vi "CalcExpress.vi"(5 "directives":T1={"enaNamedConst"=TRUE}, 7 "VC Handle":T5=-1, 8 "error in":bool, 9 "params":T3={"autoVar"=TRUE, "enCpx"=TRUE}, 10 "repeat (1)":i32=1, 11 "expression":string) -> (0 "error out":bool, 1 "value type":T4=enum."DBL Number", 2 "string value":string, 3 "numeric value":dbl, 4 "error description":string)   [LabVIEW 2021]
doc: "The VI evaluates CalcExpress expressions and sequential scripts. To process non-sequential scripts involving loops and branches, use CSE VIs.\n\n<B>VC Handle</B> should contain handle of variable context. Variables of the corresponding context can be used in an expression.\n\n<B>repeat</B> control determines number of times an expression needs to be evaluated. By default, it is equal to one (1).\n\n<B>params</B> cluster specifies optional parameters influencing on evaluation.\n params.autoVar - If it's TRUE (by default) and there is a reference to unexistent variable on the left side of an assignment operator, CalcExpress implicitly creates the variable. If it's FALSE, all variables referenced in a script must be explicitly created either before or during evaluation.\n params.enCpx parameter enables or disables performing operators on operands of non-Numeric types (TRUE by default).\n\nFor more information, see help for this VI.\n\n::: CalcExpress Toolkit :::\nCopyright (c) 2000-2026 Konstantin Shifershteyn. All rights reserved."
uses:
  cetypes.llb/VarMan Variable Context Handle.ctl
  cetypes.llb/CalcExpress Data Type.ctl
  cetypes.llb/CalcExpress Execution Options.ctl
  cetypes.llb/CalcExpress Instance RefNum.ctl
  cetypes.llb/CalcExpress Parsing Directives.ctl
  cersrc/celveng32.dll
panel:
  in  "CE InstanceRef":T2
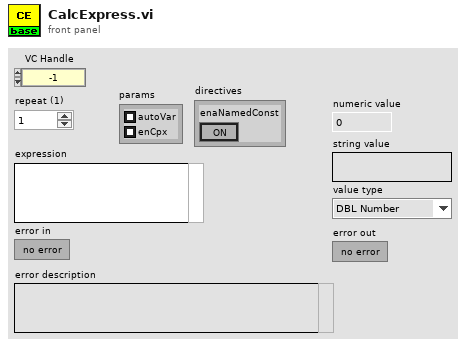
[diagram p1: front panel]
types:
  T1 = typedef "CalcExpress Parsing Directives.ctl" = cluster{"enaNamedConst":bool}
  T2 = typedef "CalcExpress Instance RefNum.ctl" = refnum<k1>
  T3 = typedef "CalcExpress Execution Options.ctl" = cluster{"autoVar":bool, "enCpx":bool}
  T4 = typedef "CalcExpress Data Type.ctl" = enum32{"String", "DBL Number", "identifier", "1D Array of DBL", "2D Array of DBL", "CDB Number", "1D Array of CDB", "2D Array of CDB", "1D Array of String", "2D Array of String", "Unknown data type"}
  T5 = typedef "VarMan Variable Context Handle.ctl" = i32
  T6 = enum32{"String", "DBL Number", "identifier", "1D Array of DBL", "2D Array of DBL", "CDB Number", "1D Array of CDB", "2D Array of CDB", "1D Array of String", "2D Array of String", "Unknown data type"}
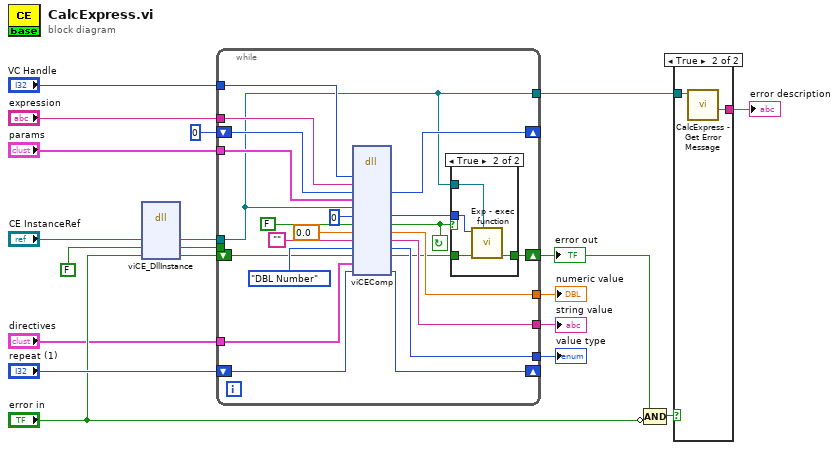
[diagram p0: block diagram]
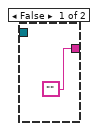
[diagram p3: hidden frame]
diagram:
  n1 = dll-call lib="C:/LV Projects/CalcExpress 40 LV2021/vi.lib/addons/CalcExpress/cersrc/celveng*.dll" fn="viCE_DllInstance"("iRef"="CE InstanceRef", "newInst"=FALSE, "err_f"="error in") -> ("iRef"=w8:T2, "newInst"=w2:bool, "err_f"=w10:bool)  [unwired: 6 in, 2 out]
  n2 = while {
    tunnel: [w21] -> w7
    shift-left: "repeat (1)" -> [w22]
    shift-right: [w23] -> _
    tunnel: [w27] -> w15
    tunnel: [w26] -> w13
    tunnel: [w28] -> w14
    tunnel: w8 -> [w21]
    tunnel: "expression" -> [w39]
    tunnel: "VC Handle" -> [w40]
    tunnel: "params" -> [w37]
    shift-left: 0 -> [w38]
    shift-right: [w31] -> _
    shift-left: w10 -> [w25]
    shift-right: [w41] -> w4
    tunnel: w2 -> [_]
    tunnel: "directives" -> [w20]
    stop <- w29 continue-if-true
    n3 = dll-call lib="C:/LV Projects/CalcExpress 40 LV2021/vi.lib/addons/CalcExpress/cersrc/celveng*.dll" fn="viCEComp"("vch"=w40, "script"=w39, "idx"=w38, "cPar"=w37, "iRef"=w21, "opdNum"=0, "NE"=FALSE, "num"=0.0, "str"="", "type"=T6."DBL Number" ("data type"), "erf"=w25, "dirs"=w20, "rept"=w22) -> ("idx"=w31:i32, "opdNum"=w30:i32, "NE"=w29:bool, "num"=w28:dbl, "str"=w27:string, "type"=w26:T6, "erf"=w24:bool, "rept"=w23:i32)  [unwired: 9 in, 2 out]
    n4 = case shown="True" w29 {
      tunnel: [w42 w46] -> w41
      tunnel: w24 -> [w42 w45]
      tunnel: w30 -> [_ w44]
      tunnel: w21 -> [_ w43]
      frame False {
      }
      frame True {
        n5 = call "Exp - exec function.vi"("CE InstanceRef"=w43, "error in"=w45, "ParNum"=w44) -> ("error out"=w46:bool)  [unwired: 6 in]
      }
    }
  }
  "error out" <- w4
  "string value" <- w15
  "numeric value" <- w14
  "value type" <- w13
  n6 = Compound Arithmetic op=AND(w4, invert "error in") -> (w3:bool)
  n7 = case shown="True" w3 {
    tunnel: w7 -> [_ w49]
    tunnel: ["" w48] -> w6
    frame False {
    }
    frame True {
      n8 = call "CalcExpress - Get Error Message.vi"("CE InstanceRef"=w49) -> ("error description"=w48:string)  [unwired: 5 in, 3 out]
    }
  }
  "error description" <- w6
